vi "images_recovery__c967ad7004.vi"(6 "interval between images (s)":dbl, 9 "Total number of images to be acquired":i32, 10 "Exposure (s)":dbl=0.0001, 11 "counter":tag) -> (1 "task done?":bool, 3 "array":cluster{dbl, dbl}[](array[cluster]))   [LabVIEW 2023]
uses:
  <vilib>/Utility/error.llb/DialogType.ctl
  <vilib>/DAQmx/write.llb/DAQmx Write (Counter 1D Time 1Chan NSamp).vi
  <vilib>/DAQmx/create/channels.llb/DAQmx Create Channel (CO-Pulse Generation-Time).vi
  <vilib>/DAQmx/configure/trigger.llb/DAQmx Start Trigger (Digital Edge).vi
  <vilib>/DAQmx/configure/timing.llb/DAQmx Timing (Implicit).vi
  <vilib>/DAQmx/miscellaneous.llb/DAQmx Fill In Error Info.vi
  <resource>/objmgr/daqmx.rc
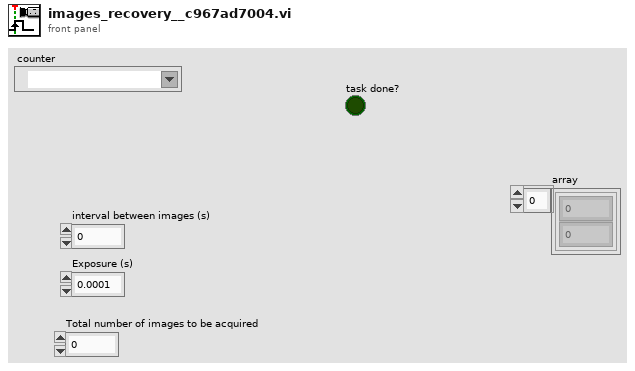
[diagram p1: front panel]
types:
  T1 = typedef "DialogType.ctl" = u16
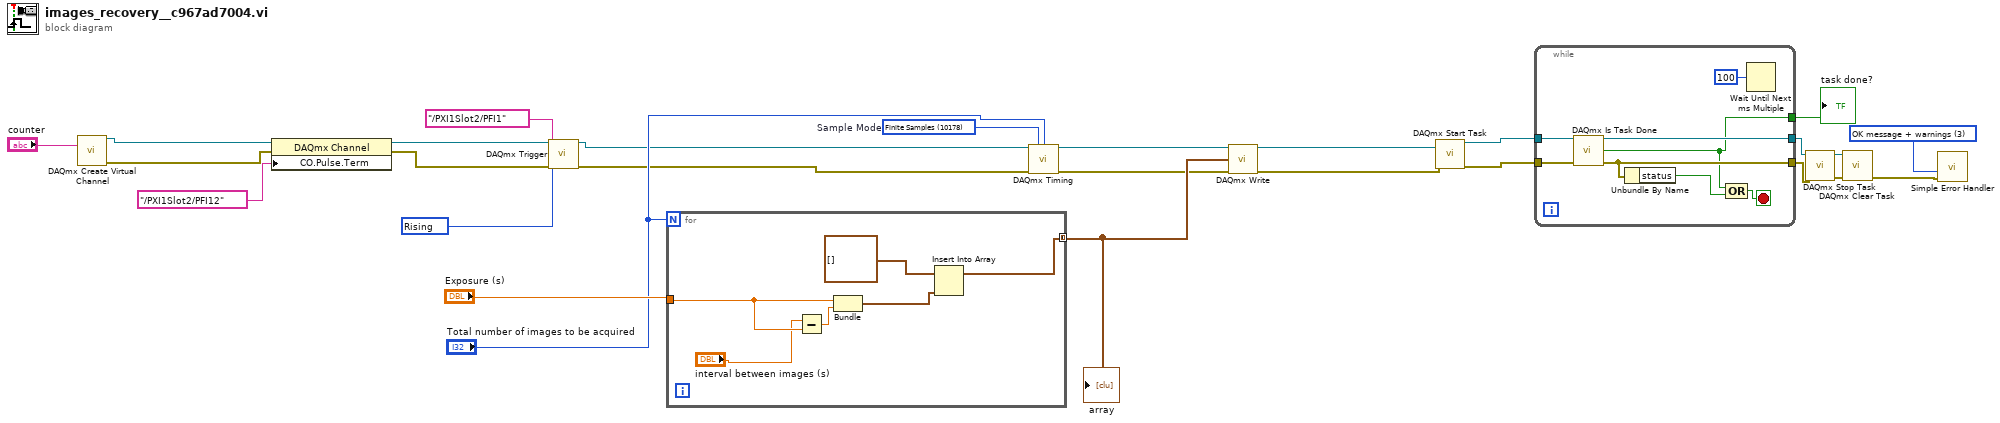
[diagram p0: block diagram]
diagram:
  w19 = 10178 items=["Finite Samples"=10178, "Continuous Samples"=10123, "Hardware Timed Single Point"=12522]  # Sample Mode
  w12 = 10280 items=["Rising"=10280, "Falling"=10171] ("edge")
  w8 = T1 3 items=["no dialog", "OK message", "continue or stop message", "OK message + warnings", "continue/stop + warnings"] ("type of dialog (OK msg:1)")
  n1 = call-poly <vilib>:"DAQmx Create Virtual Channel.vi"("counter"="counter") -> ("task out"=w20:refnum<k21>, "error out"=w21:errorcluster)  [unwired: 13 in]
  n2 = property class="DAQmx Channel"(reference=w20, error in=w21, "CO.Pulse.Term"=tag "/PXI1Slot2/PFI12") -> (reference out=w9:refnum<k21>, error out=w10:errorcluster)
  n3 = call-poly <vilib>:"DAQmx Trigger.vi"("task/channels in"=w9, "source"=tag "/PXI1Slot2/PFI1", "edge"=w12, "error in"=w10) -> ("task out"=w13:refnum<k21>, "error out"=w14:errorcluster)  [unwired: 10 in]
  n4 = for {
    N: "Total number of images to be acquired" -> [_]
    tunnel: [w33] -> w15 mode=concatenating
    tunnel: "Exposure (s)" -> [w29]
    n5 = Subtract(x="interval between images (s)", y=w29) -> (x-y=w30:dbl)
    n6 = Bundle("Exposure (s)"=w29, w30) -> (w31:cluster{"Exposure (s)":dbl, dbl})  [unwired: 1 in]
    n7 = Insert Into Array(array=cluster{dbl, dbl}[] [], new element=w31) -> (w33:cluster{dbl, dbl}[])  [unwired: 1 in]
  }
  "array" <- w15
  n8 = call-poly <vilib>:"DAQmx Timing.vi"("task/channels in"=w13, "sample mode"=w19, "samples per channel"="Total number of images to be acquired", "error in"=w14) -> ("task out"=w5:refnum<k21>, "error out"=w4:errorcluster)  [unwired: 10 in]
  n9 = call-poly <vilib>:"DAQmx Write.vi"("task/channels in"=w5, "data"=w15, "error in"=w4) -> ("task out"=w17:refnum<k21>, "error out"=w18:errorcluster)  [unwired: 10 in, 1 out]
  n10 = call <vilib>:"DAQmx Start Task.vi"("task/channels in"=w17, "error in"=w18) -> ("task out"=w23:refnum<k21>, "error out"=w22:errorcluster)  [unwired: 12 in]
  n11 = while {
    tunnel: w22 -> [w41]
    tunnel: [w38] -> w25
    tunnel: [w39] -> w24
    tunnel: w23 -> [w35]
    tunnel: [w34] -> w2
    stop <- w40 stop-if-true
    n12 = call <vilib>:"DAQmx Is Task Done.vi"("task/channels in"=w35, "error in"=w41) -> ("task out"=w39:refnum<k21>, "task done?"=w34:bool, "error out"=w38:errorcluster)  [unwired: 11 in]
    n13 = Unbundle By Name(w38) -> ("status"=w37:bool)
    n14 = Compound Arithmetic op=OR(w34, w37) -> (w40:bool)
    n15 = Wait Until Next ms Multiple(millisecond multiple=u32 100) -> ()  [unwired: 1 out]
  }
  "task done?" <- w2
  n16 = call <vilib>:"DAQmx Stop Task.vi"("task/channels in"=w24, "error in"=w25) -> ("task out"=w6:refnum<k21>, "error out"=w7:errorcluster)  [unwired: 12 in]
  n17 = call <vilib>:"DAQmx Clear Task.vi"("task in"=w6, "error in"=w7) -> ("error out"=w3:errorcluster)  [unwired: 13 in]
  n18 = call <vilib>:"Simple Error Handler.vi"("type of dialog (OK msg:1)"=w8, "error in (no error)"=w3) -> ()  [unwired: 3 in, 5 out]
